vi "RunAllTests.vi"() -> ()   [LabVIEW 2019]
uses:
  <vilib>/Utility/miscctls.llb/LVRowAndColumnUnsignedTypeDef.ctl
  ca6f43b0-97b5-4861-9fe9-a37eff1204c5.vi
  Tests.SolutionBuilder/Tests.SolutionBuilder.lvlib
  SolutionBuilder/SolutionBuilder.lvlib
panel:
  in  "Stop on Fail?":bool
  in  "Open failed tests?":bool=TRUE
  out "All Pass?":bool
  in  "Test results":i32(listbox)=-1
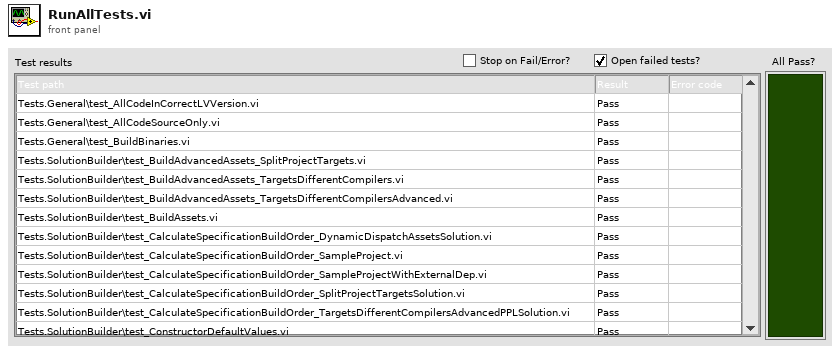
[diagram p1: front panel]
types:
  T1 = typedef "LVRowAndColumnUnsignedTypeDef.ctl" = cluster{"Row":u32, "Column":u32}
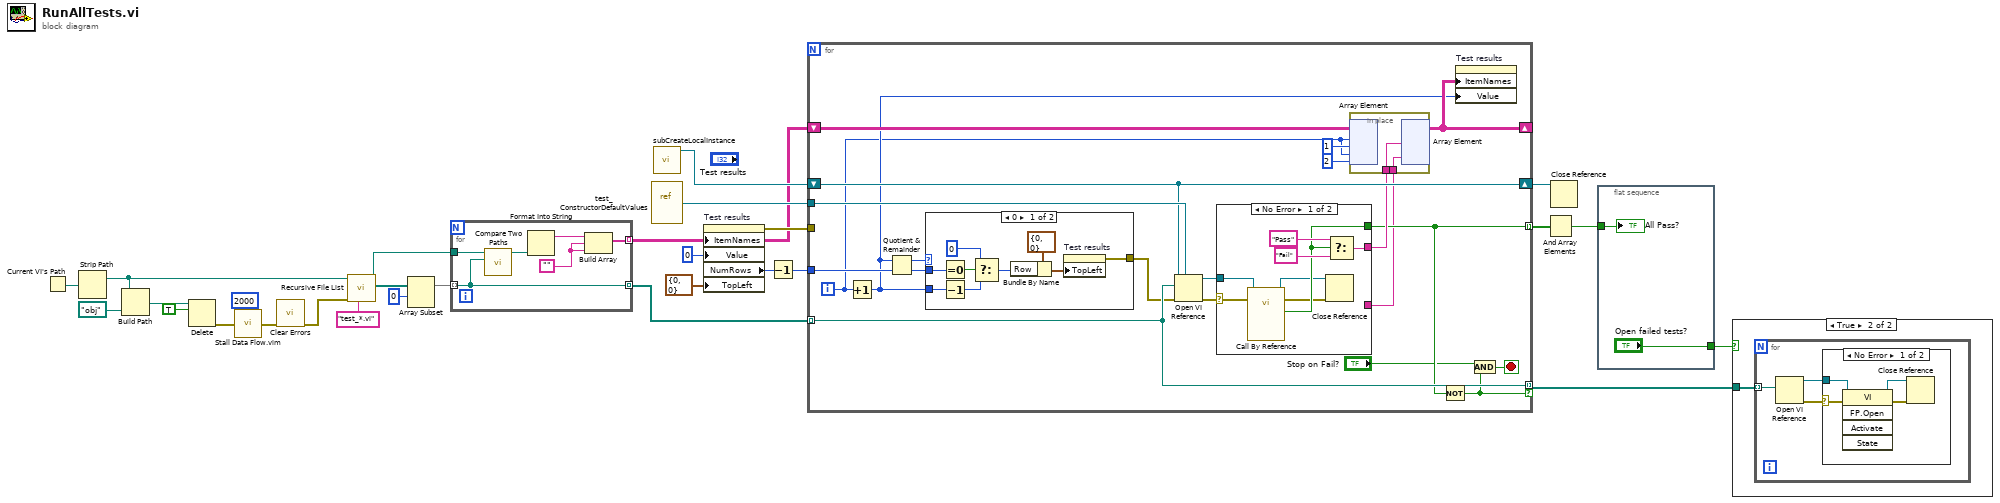
[diagram p0: block diagram]
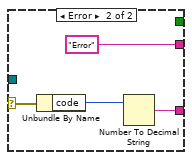
[diagram p3: hidden frame]
diagram:
  n1 = Current VI's Path() -> (path=w28:path)
  n2 = Strip Path(path=w28) -> (stripped path=w23:path)  [unwired: 1 out]
  n3 = Build Path(base path=w23, name or relative path=path "obj") -> (appended path=w21:path)
  n4 = Delete(path (use dialog)=w21, entire hierarchy (F)=TRUE) -> (error out=w19:errorcluster)  [unwired: 3 in, 2 out]
  n5 = call "Stall Data Flow.vim"("value in"=w19, "milliseconds to wait"=u32 2000) -> ("value out"=w17:errorcluster)  [unwired: 1 out]
  n6 = call <vilib>:"Clear Errors.vi"("error in (no error)"=w17) -> ("error out"=w16:errorcluster)  [unwired: 5 in, 1 out]
  n7 = call <vilib>:"Recursive File List.vi"("pattern"="test_*.vi", "error in (no error)"=w16, "Folder Path"=w23) -> ("All Files in Dir"=w6:path[], "dup Folder Path"=w13:path)  [unwired: 4 in, 3 out]
  n8 = Array Subset(array=w6, index=0) -> (w5:path[])  [unwired: 1 in]
  n9 = for {
    tunnel: w5 -> [w32] mode=indexing
    tunnel: [w32] -> w7 mode=indexing
    tunnel: w13 -> [w33]
    tunnel: [w30] -> w8 mode=indexing
    w29 = ""
    n10 = call <vilib>:"Compare Two Paths.vi"("Path 2"=w32, "Path 1"=w33) -> ("Relative Path from 1 to 2"=w34:path)  [unwired: 6 in, 3 out]
    n11 = Format Into String(w34) -> (resulting string=w31:string)  [unwired: 3 in, 1 out]
    n12 = Build Array(w31, w29, w29) -> (w30:string[])
  }
  n13 = vi-ref "test_ConstructorDefaultValues.vi"() -> (w26:refnum<vi>)
  n14 = call "subCreateLocalInstance.vi"() -> ("Application out"=w14:refnum<vi>)  [unwired: 11 in]
  n15 = property on="Test results" class="MCListbox (strict)"("ItemNames"=w8, "Value"=0 ("Test results"), "TopLeft"=T1 {"Row"=0, "Column"=0} ("Top Left Visible Cell")) -> (error out=w11:errorcluster, "NumRows"=w3:u32)  [unwired: 2 in, 1 out]
  n16 = Decrement(x=w3) -> (x-1=w1:u32)
  n17 = for {
    tunnel: w7 -> [w47] mode=indexing
    tunnel: w26 -> [w55]
    tunnel: [w46] -> w25 mode=indexing
    shift-right: [w52] -> w15
    shift-left: w14 -> [w52]
    tunnel: w11 -> [_]
    shift-right: [w48] -> _
    shift-left: w8 -> [w51]
    tunnel: [w47] -> w9 mode=indexing if=w45
    tunnel: w1 -> [w38]
    i -> [w36]
    stop <- w44 stop-if-true
    n18 = Increment(x=w36) -> (x+1=w37:i32)
    n19 = Quotient & Remainder(x=w37, y=w38) -> (x-y*floor(x/y)=w40:u32, floor(x/y)=w39:u32)
    n20 = case shown="0" w40 {
      tunnel: w39 -> [w62 _]
      tunnel: w37 -> [w58 _]
      tunnel: [w56 _] -> w35
      frame 0 {
        n21 = Equal To 0?(x=w62) -> (x = 0?=w61:bool)
        n22 = Decrement(x=w58) -> (x-1=w57:i32)
        n23 = Select(t=u32 0 ("Row"), s=w61, f=w57) -> (s? t:f=w59:u32)
        n24 = Bundle By Name(cluster=T1 {"Row"=0, "Column"=0} ("Top Left Visible Cell"), "Row"=w59) -> (w63:T1)
        n25 = property on="Test results" class="MCListbox (strict)"("TopLeft"=w63) -> (error out=w56:errorcluster)  [unwired: 2 in, 1 out]
      }
      frame Default {
      }
    }
    n26 = Open VI Reference(type specifier VI Refnum (for type only)=w55, application reference (local)=w52, vi path=w47, error in (no error)=w35) -> (vi reference=w54:refnum<vi>, error out=w53:errorcluster)  [unwired: 2 in]
    n27 = case shown="No Error" w53 {
      selector: w53 -> [w71 w77]
      tunnel: w54 -> [w74 _]
      tunnel: [w69 "Error" ("resulting string")] -> w49
      tunnel: [w70 _] -> w46
      tunnel: [_ w75] -> w41
      frame No Error {
        n28 = call-by-ref "?"(reference=w74, error in=w71) -> (reference out=w67:refnum<vi>, error out=w68:errorcluster, "Pass?"=w70:bool)  [unwired: 11 in]
        n29 = Close Reference(reference=w67, error in (no error)=w68) -> ()  [unwired: 1 out]
        n30 = Select(t="Pass" ("resulting string"), s=w70, f="Fail" ("resulting string")) -> (s? t:f=w69:string)
      }
      frame Error {
        n31 = Unbundle By Name(w77) -> ("code"=w76:i32)
        n32 = Number To Decimal String(number=w76) -> (decimal integer string=w75:string)  [unwired: 1 in]
      }
    }
    n33 = in-place {
      in-place-border: w49 -> [w66]
      in-place-border: w41 -> [w65]
      n34 = in-place-array #1(w51, w36, 1, w36, 2) -> ()  [unwired: 2 out]
      n35 = in-place-array #1(w66, w65) -> (w48:string[][])  [unwired: 4 out]
    }
    n36 = Not(x=w46) -> (.not. x?=w45:bool)
    n37 = property on="Test results" class="MCListbox (strict)"("ItemNames"=w48, "Value"=w37) -> ()  [unwired: 2 in, 2 out]
    n38 = And(x="Stop on Fail?", y=w45) -> (x .and. y?=w44:bool)
  }
  n39 = And Array Elements(Boolean array=w25) -> (logical AND=w24:bool)
  n40 = Close Reference(reference=w15) -> ()  [unwired: 1 in, 1 out]
  n41 = flat-sequence {
    tunnel: w24 -> [w80]
    tunnel: ["Open failed tests?"] -> w10
    frame #0 {
      "All Pass?" <- w80
    }
  }
  n42 = case shown="True" w10 {
    tunnel: w9 -> [_ w81]
    frame False {
    }
    frame True {
      n43 = for {
        tunnel: w81 -> [w82] mode=indexing
        n44 = Open VI Reference(vi path=w82) -> (vi reference=w84:refnum<vi>, error out=w83:errorcluster)  [unwired: 5 in]
        n45 = case shown="No Error" w83 {
          selector: w83 -> [w87 _]
          tunnel: w84 -> [w88 _]
          frame No Error {
            n46 = invoke class="VI" method="FP.Open"(reference=w88, error in=w87) -> (reference out=w85:refnum<vi>, error out=w86:errorcluster)  [unwired: 3 in, 3 out]
            n47 = Close Reference(reference=w85, error in (no error)=w86) -> ()  [unwired: 1 out]
          }
          frame Error {
          }
        }
      }
    }
  }
